vi "Get MSE.vi"(7 "Color":T1, 10 "y (lux)":dbl[](array[numeric]), 11 "x (volts)":dbl[](array[numeric])) -> (3 "MSE":dbl)   [LabVIEW 2020]
uses:
  controls/Color --typedef.ctl
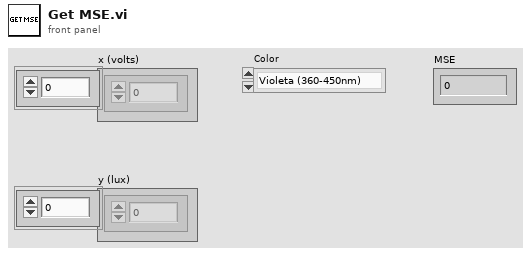
[diagram p1: front panel]
types:
  T1 = typedef "Color --typedef.ctl" = enum16{"Violeta (360-450nm)", "Azul (450-500nm)", "Verde(500-570nm)", "Amarillo (570-590nm)", "Naranja (600-610nm)", "Rojo (610-670nm)", "Blanco"}
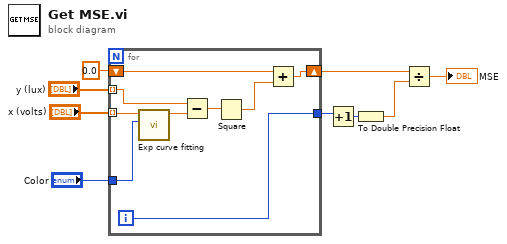
[diagram p0: block diagram]
diagram:
  n1 = for {
    tunnel: "x (volts)" -> [w18] mode=indexing
    tunnel: "y (lux)" -> [w15] mode=indexing
    tunnel: "Color" -> [w17]
    shift-right: [w12] -> w5
    shift-left: 0.0 -> [w11]
    tunnel: [w10] -> w4
    i -> [w10]
    n2 = call "Exp curve fitting.vi"("Color"=w17, "x (volts)"=w18) -> ("y (Lux)"=w16:dbl)  [unwired: 9 in]
    n3 = Subtract(x=w15, y=w16) -> (x-y=w14:dbl)
    n4 = Square(x=w14) -> (x^2=w13:dbl)
    n5 = Add(x=w11, y=w13) -> (x+y=w12:dbl)
  }
  n6 = Increment(x=w4) -> (x+1=w3:i32)
  n7 = To Double Precision Float(number=w3) -> (double precision float=w2:dbl)
  n8 = Divide(x=w5, y=w2) -> (x/y=→"MSE":dbl)
